vi "Group Exists.vi"(4 "error in (no error)":errorcluster, 6 "Group Name":string, 7 "EasyUserManager in":refnum<class "EasyUserManager.lvclass">) -> (0 "error out":errorcluster, 2 "Group Exists":bool, 3 "EasyUserManager out":refnum<class "EasyUserManager.lvclass">)   [LabVIEW 2024, in "EasyUserManager.lvclass"]
doc: "Check if the group specified by <B>Group Name</B> exists in the list of user groups."
uses:
  EasyUserManager.lvclass
  EasyUserManager.lvclass/EasyUserManager.ctl
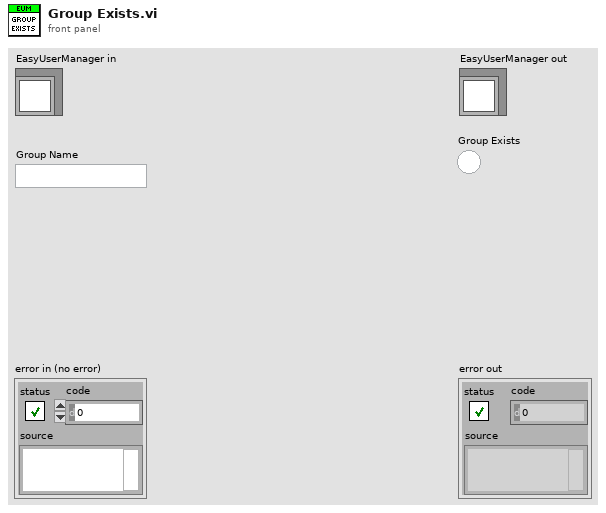
[diagram p1: front panel]
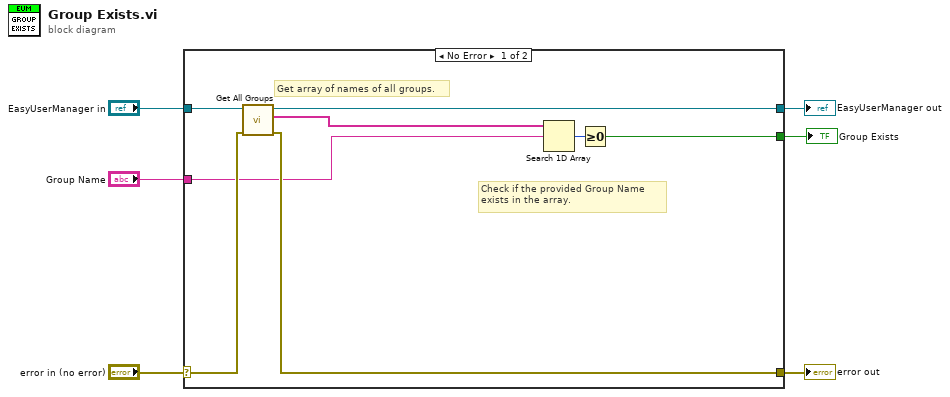
[diagram p0: block diagram]
diagram:
  n1 = case shown="No Error" "error in (no error)" {
    selector: "error in (no error)" -> [w12 w16]
    tunnel: [w11 w16] -> w5
    tunnel: [w14 w15] -> w3
    tunnel: "EasyUserManager in" -> [w13 w15]
    tunnel: "Group Name" -> [w8 _]
    tunnel: [w7 _] -> w1
    frame No Error {
      # "Check if the provided Group Name\nexists in the array."
      # "Get array of names of all groups."
      n2 = call "Get All Groups.vi"("error in (no error)"=w12, "EasyUserManager in"=w13) -> ("error out"=w11:errorcluster, "Groups"=w10:string[], "EasyUserManager out"=w14:refnum<class "EasyUserManager.lvclass">)  [unwired: 3 in]
      n3 = Search 1D Array(1D array=w10, element=w8) -> (index of element=w9:i32)  [unwired: 1 in]
      n4 = Greater Or Equal To 0?(x=w9) -> (x >= 0?=w7:bool)
    }
    frame Error {
      # "Pass error and do nothing."
    }
  }
  "error out" <- w5
  "EasyUserManager out" <- w3
  "Group Exists" <- w1
